vi "FuncVI_Sub - File - Base Path.vi"(5 "InstanceRef":T1, 6 "error in":bool, 7 "cmd":enum16{"get", "set"}(ring), 9 "str arg: path":string) -> (0 "error out":bool, 2 "base path":path, 3 "path str":string)   [LabVIEW 2021]
doc: "::: CalcExpress Toolkit :::\nCopyright (c) 2000-2026 Konstantin Shifershteyn. All rights reserved."
uses:
  cetypes.llb/CalcExpress Instance RefNum.ctl
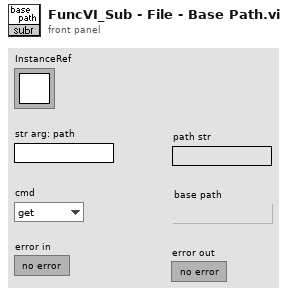
[diagram p1: front panel]
types:
  T1 = typedef "CalcExpress Instance RefNum.ctl" = refnum<k1>
  T2 = typedef "VarMan Variable Context Handle.ctl" = i32
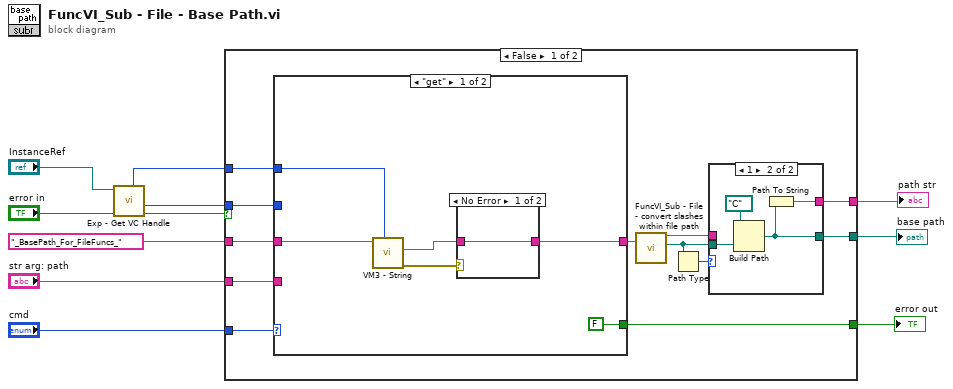
[diagram p0: block diagram]
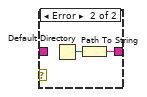
[diagram p3: hidden frame]
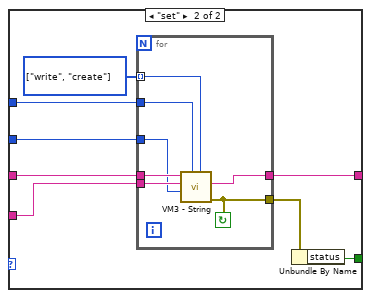
[diagram p4: hidden frame]
diagram:
  n1 = call "Exp - Get VC Handle.vi"("error in"="error in", "InstanceRef"="InstanceRef") -> ("error out"=w2:bool, "writer ID"=w1:u32, "VC Handle"=w9:T2)  [unwired: 4 in, 1 out]
  n2 = case shown="False" w2 {
    selector: w2 -> [_ w54]
    tunnel: "cmd" -> [w23 _]
    tunnel: "_BasePath_For_FileFuncs_" -> [w22 _]
    tunnel: w9 -> [w21 _]
    tunnel: [w20 w54] -> w6
    tunnel: [w16 _] -> w5
    tunnel: [w15 _] -> w4
    tunnel: "str arg: path" -> [w13 _]
    tunnel: w1 -> [w12 _]
    frame False {
      n3 = case shown="\"get\"" w23 {
        tunnel: w22 -> [w32 w46]
        tunnel: w21 -> [w31 w43]
        tunnel: [w35 w45] -> w19
        tunnel: [FALSE ("error out") w39] -> w20
        tunnel: w13 -> [_ w44]
        tunnel: w12 -> [_ w42]
        frame "get" {
          n4 = call "VM3 - String.vi"("VC Handle"=w31, "name_spec"=w32) -> ("error out"=w33:errorcluster, "value out"=w30:string)  [unwired: 6 in, 2 out]
          n5 = case shown="No Error" w33 {
            tunnel: w30 -> [w36 _]
            tunnel: [w36 w37] -> w35
            frame No Error {
            }
            frame Error {
              n6 = Default Directory() -> (w38:path)
              n7 = Path To String(path=w38) -> (string=w37:string)
            }
          }
        }
        frame "set" {
          w41 = enum16{"create", "destroy", "write", "read"}[] [enum."write", enum."create"] items=["create", "destroy", "write", "read"]
          n8 = for {
            tunnel: [w49] -> w45
            tunnel: w44 -> [w51]
            tunnel: w46 -> [w52]
            tunnel: w43 -> [w53]
            tunnel: w42 -> [w50]
            tunnel: w41 -> [w48] mode=indexing
            tunnel: [w47] -> w40
            stop <- w47 continue-if-true
            n9 = call "VM3 - String.vi"("cmd (read)"=w48, "VC Handle"=w53, "writer ID"=w50, "value in"=w51, "name_spec"=w52) -> ("error out"=w47:errorcluster, "value out"=w49:string)  [unwired: 3 in, 2 out]
          }
          n10 = Unbundle By Name(w40) -> ("status"=w39:bool)
        }
      }
      n11 = call "FuncVI_Sub - File - convert slashes within file path.vi"("str: path"=w19) -> ("str: path out"=w14:string, "path out"=w17:path)  [unwired: 3 in]
      n12 = Path Type(1:w17) -> (0:w18:i16)
      n13 = case shown="1" w18 {
        tunnel: w17 -> [w25 w29]
        tunnel: [w25 w27] -> w16
        tunnel: [w24 w26] -> w15
        tunnel: w14 -> [w24 _]
        frame 0, Default {
        }
        frame 1 {
          n14 = Build Path(base path=path "C:/", name or relative path=w29) -> (appended path=w27:path)
          n15 = Path To String(path=w27) -> (string=w26:string)
        }
      }
    }
    frame True {
    }
  }
  "base path" <- w5
  "error out" <- w6
  "path str" <- w4
